vi "Tableau en chaine.vi"(2 "error in (no error)":errorcluster caption="entrée d'erreur (pas d'erreur)", 3 "Tableau 1D":string[](array[string])) -> (0 "error out":errorcluster caption="sortie d'erreur", 1 "Chaîne":string)   [LabVIEW 2022 SP3]
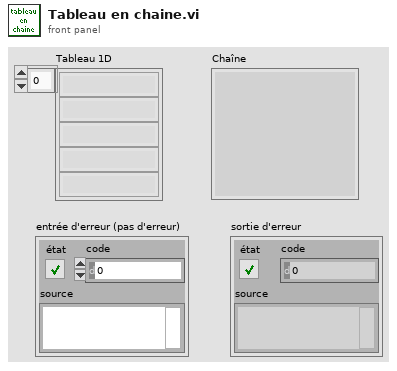
[diagram p1: front panel]
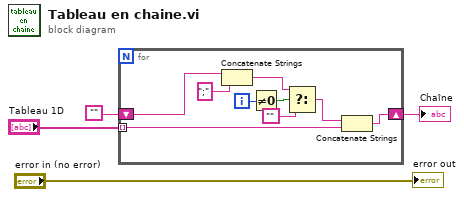
[diagram p0: block diagram]
diagram:
  n1 = for {
    tunnel: "Tableau 1D" -> [w13] mode=indexing
    shift-right: [w5] -> w4
    shift-left: "" -> [w10]
    i -> [w12]
    n2 = Concatenate Strings(w10, ";" ("chaîne")) -> (w8:string)
    n3 = Not Equal To 0?(x=w12) -> (x != 0?=w11:bool)
    n4 = Select(t=w8, s=w11, f="") -> (s? t:f=w7:string)
    n5 = Concatenate Strings(w7, w13) -> (w5:string)
  }
  "Chaîne" <- w4
  "error out" <- "error in (no error)"
